vi "Parse State Queue_csmlite.vi"(0 "State Queue":string, 1 "Current Module(\"\" to generate an ID)":string="Debug-LogViewer", 7 "Error In (no error)":errorcluster) -> (3 "Event Registration Refnum":refnum<event-registration>, 4 "Remaining States":string, 6 "Current State":string, 8 "Arguments":string)   [LabVIEW 2017, in "_csmlite.lvlib"]
doc: "Parses the JKI State Machine state queue and returns the current state that will execute next with the associated arguments."
uses:
  _csmlite.lvlib
  _action.ctl
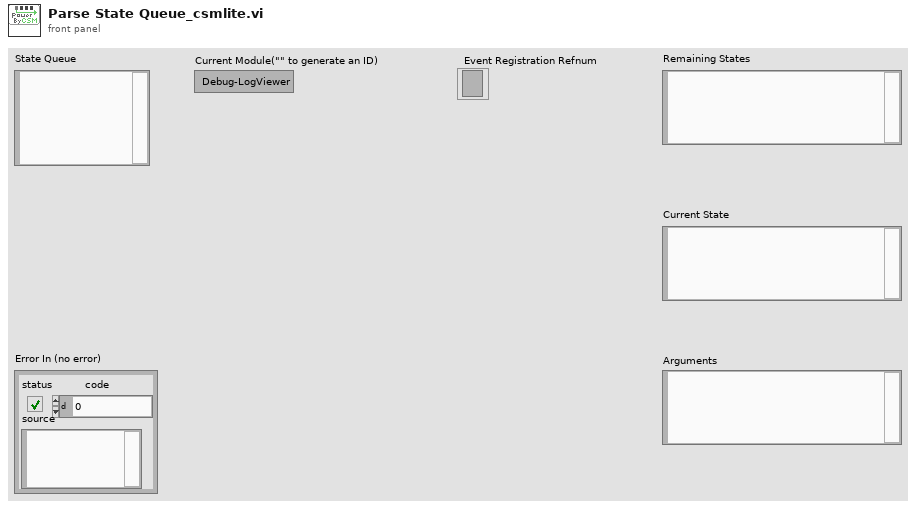
[diagram p1: front panel]
types:
  T1 = typedef "_csmlite.lvlib/_action.ctl" = enum16{"Obtain", "Destroy", "Broadcast", "Post", "List"}
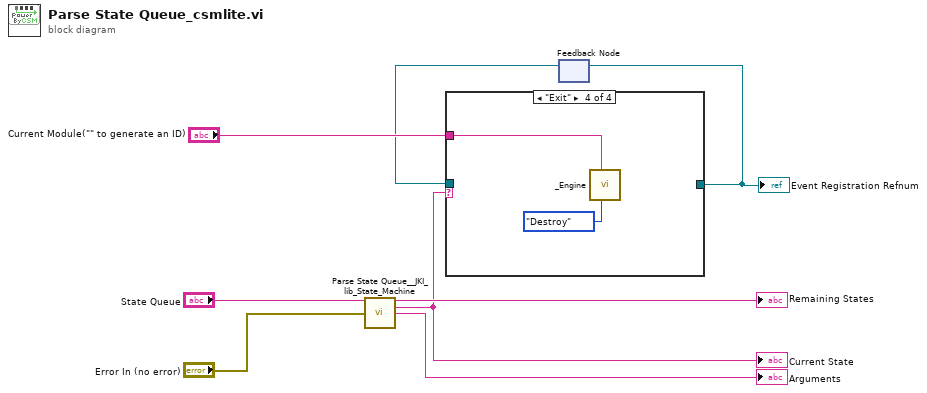
[diagram p0: block diagram]
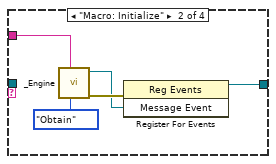
[diagram p3: hidden frame]
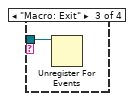
[diagram p4: hidden frame]
diagram:
  n1 = call <vilib>:"Parse State Queue__JKI_lib_State_Machine.vi"("State Queue"="State Queue", "Error In (no error)"="Error In (no error)") -> ("Remaining States"=→"Remaining States":string, "Current State"=w3:string, "Arguments"=→"Arguments":string)  [unwired: 11 in]
  "Current State" <- w3
  n2 = feedback #1() -> (w2:refnum<event-registration>)  [unwired: 1 in]
  n3 = case shown="\"Exit\"" w3 {
    tunnel: "Current Module(\"\" to generate an ID)" -> [_ w12 _ w16]
    tunnel: [w9 w11 _ _] -> w1
    tunnel: w2 -> [w9 _ w15 _]
    frame "False", Default {
    }
    frame "Macro: Initialize" {
      n4 = call "_Engine.vi"("Enum"=_action."Obtain", "Module Name"=w12) -> ("Error out"=w14:errorcluster, "Message Event"=w10:refnum<user-event>)  [unwired: 7 in, 1 out]
      n5 = register-events(error in=w14, w10) -> (reference out=w11:refnum<event-registration>)  [unwired: 1 in, 1 out]
    }
    frame "Macro: Exit" {
      n6 = Unregister For Events(event registration refnum=w15) -> ()  [unwired: 1 in, 1 out]
    }
    frame "Exit" {
      n7 = call "_Engine.vi"("Enum"=_action."Destroy", "Module Name"=w16) -> ()  [unwired: 7 in, 3 out]
    }
  }
  "Event Registration Refnum" <- w1
  n8 = feedback-in #1(w1) -> ()
